vi "SMS Candidate Selection.vi"(0 "Image Ref (U16)":T1, 7 "Blink Sensitivity":sgl=1.3, 11 "Error In":errorcluster) -> (4 "Image Ref (U16) - Dup":T1, 8 "Cadidate Image Ref":T1, 15 "Error Out":errorcluster)   [LabVIEW 2021]
uses:
  <vilib>/vision/Image Controls.llb/IMAQ Image.ctl
  Microscope Modules/SMS Image Preview/SMS Image Preview Type Defs/SMS Image Preview Actions.ctl
  <vilib>/vision/NI_Vision_Development_Module.lvlib
panel:
  out "Image border size out":i32
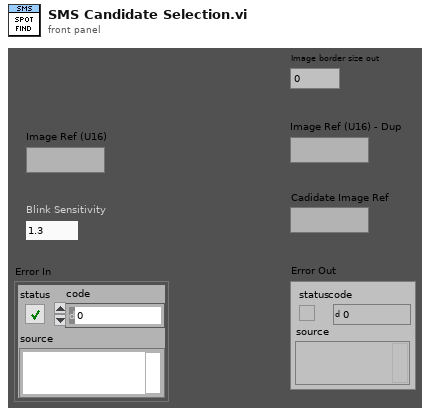
[diagram p1: front panel]
types:
  T1 = typedef "IMAQ Image.ctl" = refnum<image>
  T2 = typedef "Image Type" = u32
  T3 = enum32{"Average", "Min", "Max", "Clear  if < ", "Clear  if < or =", "Clear  if =", "Clear  if > or =", "Clear  if >"}
  T4 = enum32{"AutoM", "Close", "Dilate", "Erode", "Gradient", "Gradient in", "Gradient out", "HitMiss", "Open", "PClose", "POpen", "Thick", "Thin"}
  T5 = cluster{"histogram":u32[], "Minimal Value":sgl, "Maximal Value":sgl, "Starting Value":sgl, "Interval Width":sgl, "Mean Value":sgl, "Standard  Variation":sgl, "Area (pixels)":i32}
  T6 = typedef "SMS Image Preview Actions.ctl" = enum16{"Idle", "Start SMS Preview", "Get Image", "Convolve and Threshold", "Subtract > Dilate", "And Image", "Update Plot", "Abort", "Exit Loop", "Quit"}
  T7 = typedef "SMS Image Preview Notifier Type.ctl" = cluster{"Action":T6, "Camera Notifier Name":string, "Camera Image (U16)":T1, "Camera ROI":cluster{"Global Rectangle":i32[], "Contours":cluster{"Contour Type":u32, "ROI Type":u32, "Points":i32[]}[]}, "SMS Preview (U16)":T1, "Camera ROI (U16)":T1, "Threshold (U16)":T1, "Subtracted > Dilated (U16)":T1, "And Image (U16)":T1, "Camera ROI (SGL)":T1, "Conv 5 x 5 (SGL)":T1, "Conv 11 x 11 (SGL)":T1, "Subtracted (SGL)":T1, "Dilated (SGL)":T1, "Subtracted > Dilated (SGL)":T1, "Ones 5 x 5":sgl[][], "Ones 11 x 11":sgl[][], "Ones 7 x 7":i32[][]}
  T8 = cluster{"Global Rectangle":i32[], "Contours":cluster{"Contour Type":u32, "ROI Type":u32, "Points":i32[]}[]}
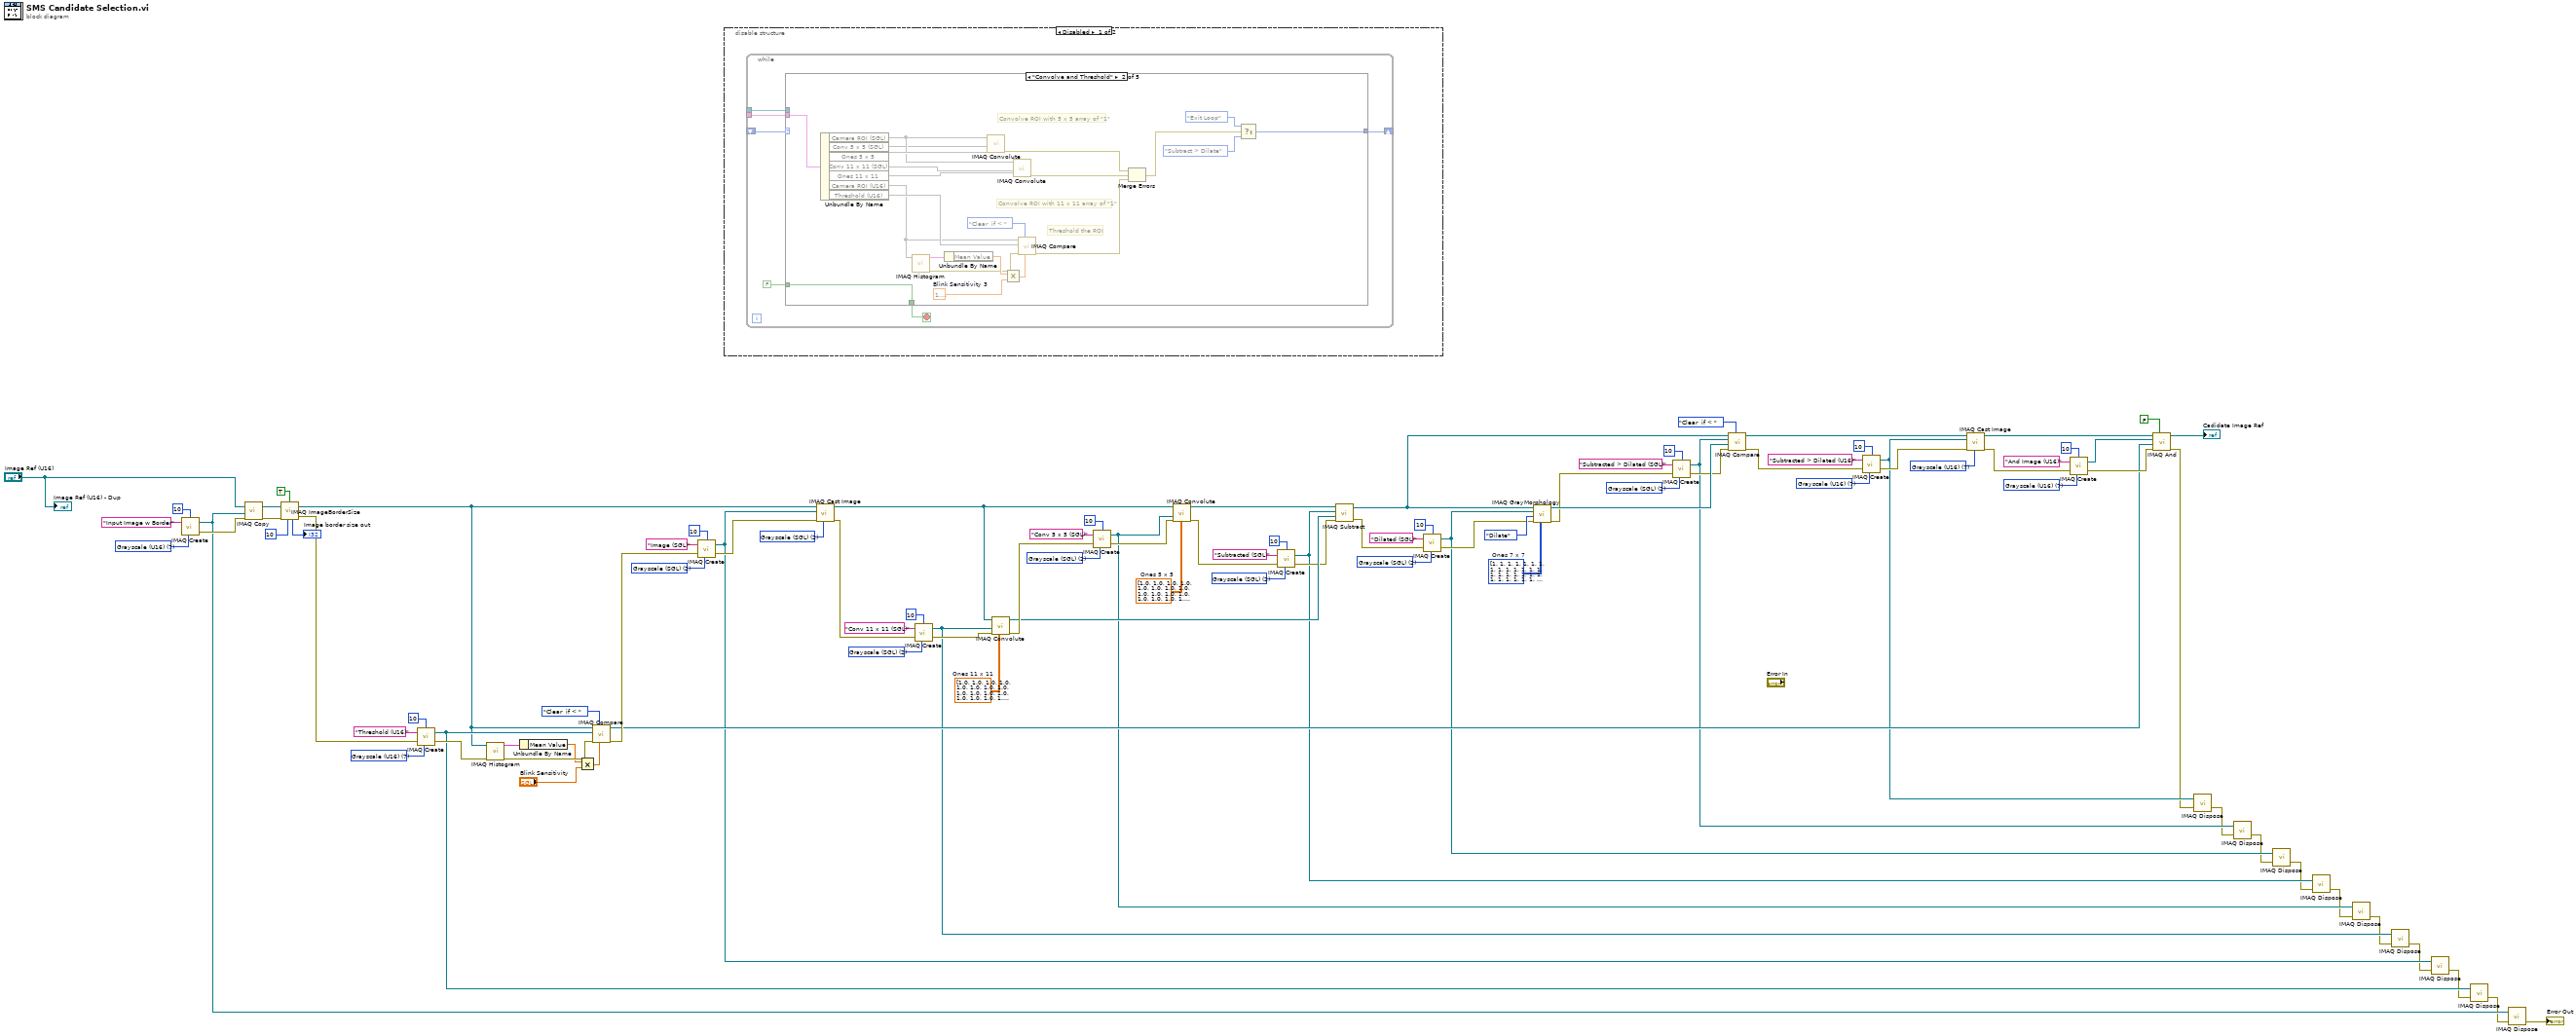
[diagram p0: block diagram]
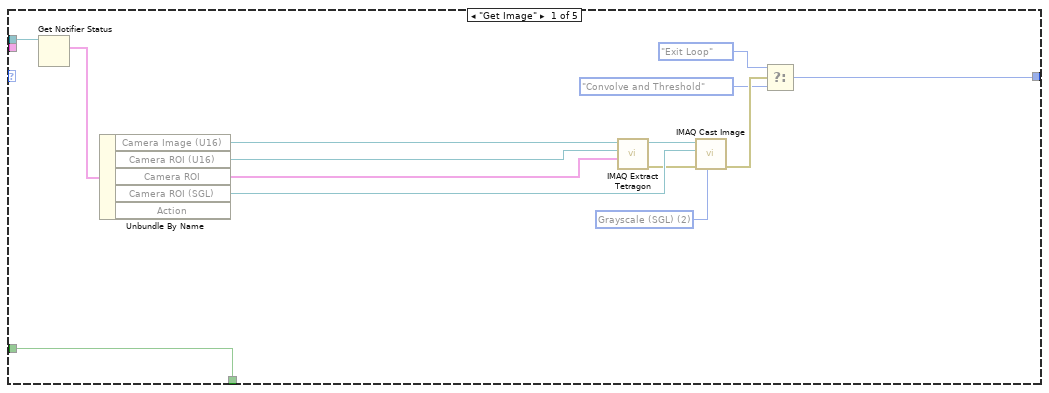
[diagram p2: hidden frame]
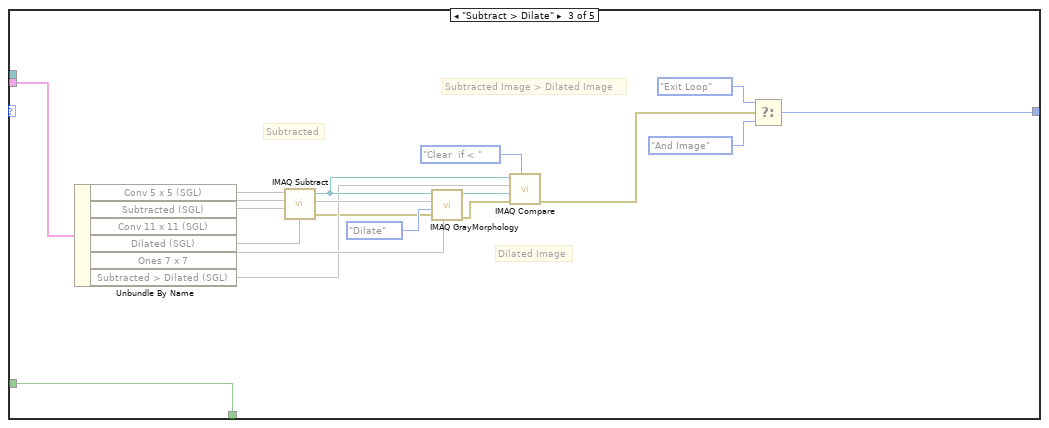
[diagram p3: hidden frame]
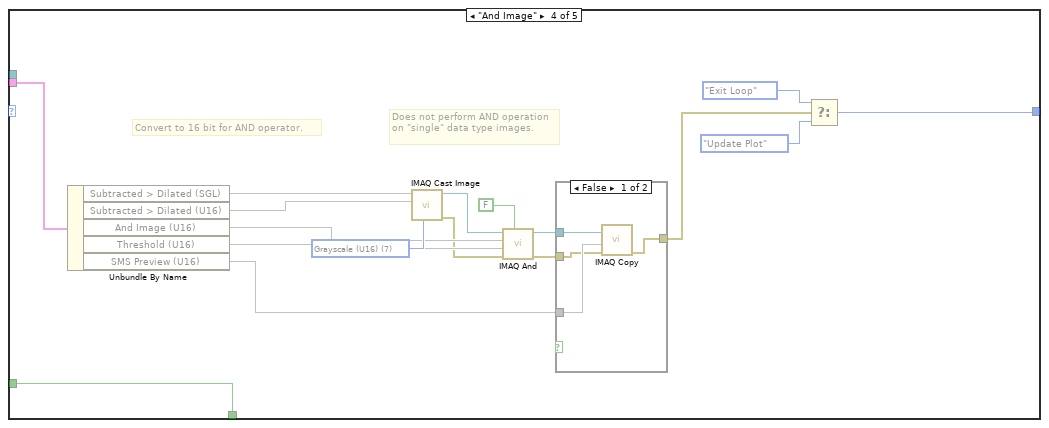
[diagram p4: hidden frame]
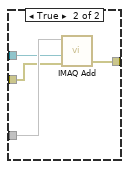
[diagram p5: hidden frame]
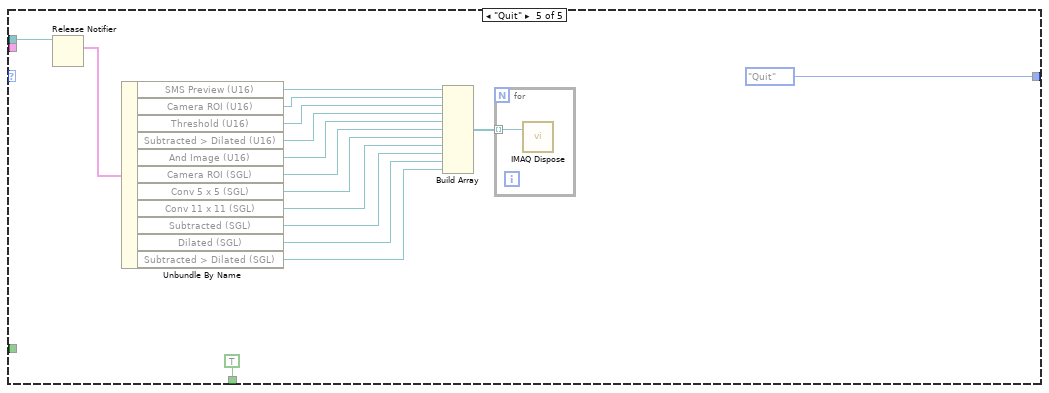
[diagram p6: hidden frame]
diagram:
  w15 = T2 7 items=["Grayscale (U8)", "Grayscale (I16)", "Grayscale (SGL)", "Complex (CSG)", "RGB (U32)", "HSL (U32)", "RGB (U64)", "Grayscale (U16)"] ("Image Type")
  w38 = T2 7 items=["Grayscale (U8)", "Grayscale (I16)", "Grayscale (SGL)", "Complex (CSG)", "RGB (U32)", "HSL (U32)", "RGB (U64)", "Grayscale (U16)"] ("Image Type")
  w48 = T2 7 items=["Grayscale (U8)", "Grayscale (I16)", "Grayscale (SGL)", "Complex (CSG)", "RGB (U32)", "HSL (U32)", "RGB (U64)", "Grayscale (U16)"] ("Image Type")
  w50 = T2 7 items=["Grayscale (U8)", "Grayscale (I16)", "Grayscale (SGL)", "Complex (CSG)", "RGB (U32)", "HSL (U32)", "RGB (U64)", "Grayscale (U16)"] ("Image Type")
  w53 = T2 2 items=["Grayscale (U8)", "Grayscale (I16)", "Grayscale (SGL)", "Complex (CSG)", "RGB (U32)", "HSL (U32)", "RGB (U64)", "Grayscale (U16)"] ("Image Type")
  w59 = i32[][] [[1, 1, 1, 1, 1, 1, 1], [1, 1, 1, 1, 1, 1, 1], [1, 1, 1, 1, 1, 1, 1], [1, 1, 1, 1, 1, 1, 1], [1, 1, 1, 1, 1, 1, 1], [1, 1, 1, 1, 1, 1, 1], [1, 1, 1, 1, 1, 1, 1]]  # Ones 7 x 7
  w63 = T2 2 items=["Grayscale (U8)", "Grayscale (I16)", "Grayscale (SGL)", "Complex (CSG)", "RGB (U32)", "HSL (U32)", "RGB (U64)", "Grayscale (U16)"] ("Image Type")
  w72 = T2 2 items=["Grayscale (U8)", "Grayscale (I16)", "Grayscale (SGL)", "Complex (CSG)", "RGB (U32)", "HSL (U32)", "RGB (U64)", "Grayscale (U16)"] ("Image Type")
  w79 = T2 7 items=["Grayscale (U8)", "Grayscale (I16)", "Grayscale (SGL)", "Complex (CSG)", "RGB (U32)", "HSL (U32)", "RGB (U64)", "Grayscale (U16)"] ("Image Type")
  w89 = T2 2 items=["Grayscale (U8)", "Grayscale (I16)", "Grayscale (SGL)", "Complex (CSG)", "RGB (U32)", "HSL (U32)", "RGB (U64)", "Grayscale (U16)"] ("Image Type")
  w90 = T2 2 items=["Grayscale (U8)", "Grayscale (I16)", "Grayscale (SGL)", "Complex (CSG)", "RGB (U32)", "HSL (U32)", "RGB (U64)", "Grayscale (U16)"] ("Image Type")
  w93 = sgl[][] [[1.0, 1.0, 1.0, 1.0, 1.0, 1.0, 1.0, 1.0, 1.0, 1.0, 1.0], [1.0, 1.0, 1.0, 1.0, 1.0, 1.0, 1.0, 1.0, 1.0, 1.0, 1.0], [1.0, 1.0, 1.0, 1.0, 1.0, 1.0, 1.0, 1.0, 1.0, 1.0, 1.0], [1.0, 1.0, 1.0, 1.0, 1.0, 1.0, 1.0, 1.0, 1.0, 1.0, 1.0], [1.0, 1.0, 1.0, 1.0, 1.0, 1.0, 1.0, 1.0, 1.0, 1.0, 1.0], [1.0, 1.0, 1.0, 1.0, 1.0, 1.0, 1.0, 1.0, 1.0, 1.0, 1.0], [1.0, 1.0, 1.0, 1.0, 1.0, 1.0, 1.0, 1.0, 1.0, 1.0, 1.0], [1.0, 1.0, 1.0, 1.0, 1.0, 1.0, 1.0, 1.0, 1.0, 1.0, 1.0], [1.0, 1.0, 1.0, 1.0, 1.0, 1.0, 1.0, 1.0, 1.0, 1.0, 1.0], [1.0, 1.0, 1.0, 1.0, 1.0, 1.0, 1.0, 1.0, 1.0, 1.0, 1.0], [1.0, 1.0, 1.0, 1.0, 1.0, 1.0, 1.0, 1.0, 1.0, 1.0, 1.0]]  # Ones 11 x 11
  w94 = sgl[][] [[1.0, 1.0, 1.0, 1.0, 1.0], [1.0, 1.0, 1.0, 1.0, 1.0], [1.0, 1.0, 1.0, 1.0, 1.0], [1.0, 1.0, 1.0, 1.0, 1.0], [1.0, 1.0, 1.0, 1.0, 1.0]]  # Ones 5 x 5
  w98 = T2 2 items=["Grayscale (U8)", "Grayscale (I16)", "Grayscale (SGL)", "Complex (CSG)", "RGB (U32)", "HSL (U32)", "RGB (U64)", "Grayscale (U16)"] ("Image Type")
  w99 = T2 2 items=["Grayscale (U8)", "Grayscale (I16)", "Grayscale (SGL)", "Complex (CSG)", "RGB (U32)", "HSL (U32)", "RGB (U64)", "Grayscale (U16)"] ("Image Type")
  n1 = call "IMAQ Create"("Border Size"=10, "Image Name"="Input Image w Border", "Image Type"=w15) -> ("New Image"=w10:T1, "error out"=w12:errorcluster)  [unwired: 2 in]
  n2 = call "IMAQ Copy"("error in (no error)"=w12, "Image Dst"=w10, "Image Src"="Image Ref (U16)") -> ("error out"=w3:errorcluster, "Image Dst Out"=w7:T1)  [unwired: 3 in]
  n3 = call "IMAQ ImageBorderSize"("Get/Set Status? (Set)"=TRUE, "Image"=w7, "Image border size in"=10, "error in (no error)"=w3) -> ("Image Out"=w5:T1, "error out"=w2:errorcluster, "Image border size out"=→"Image border size out":i32)
  n4 = call "IMAQ Create"("Border Size"=10, "Image Name"="Threshold (U16)", "Image Type"=w79, "error in (no error)"=w2) -> ("New Image"=w32:T1, "error out"=w40:errorcluster)  [unwired: 1 in]
  n5 = call "IMAQ Histogram"("error in (no error)"=w40, "Image"=w5) -> ("error out"=w78:errorcluster, "Histogram Report"=w75:T5)  [unwired: 8 in]
  n6 = Unbundle By Name(w75) -> ("Mean Value"=w74:sgl)
  n7 = Multiply(x=w74, y="Blink Sensitivity") -> (x*y=w73:sgl)
  n8 = call "IMAQ Compare"("Constant"=w73, "Operator"=T3."Clear  if < ", "error in (no error)"=w78, "Image Dst"=w32, "Image Src A"=w5) -> ("error out"=w41:errorcluster, "Image Dst Out"=w34:T1)  [unwired: 5 in]
  n9 = call "IMAQ Create"("Border Size"=10, "Image Name"="Image (SGL)", "Image Type"=w98, "error in (no error)"=w41) -> ("New Image"=w31:T1, "error out"=w83:errorcluster)  [unwired: 1 in]
  n10 = disable-structure shown="Disabled" {
    frame Disabled {
      n11 = while {
        shift-right: [w103] -> _
        shift-left: _ -> [w105]
        tunnel: _ -> [w104]
        tunnel: _ -> [w102]
        stop <- w100 stop-if-true
        n12 = case shown="\"Convolve and Threshold\"" w105 {
          tunnel: w104 -> [_ w141 w159 w176 _]
          tunnel: [w110 w122 w142 w160 SMS_Image_Preview_Actions."Quit" ("f")] -> w103
          tunnel: w102 -> [w115 _ _ _ w198]
          tunnel: FALSE -> [w116 w132 w148 w166 _]
          tunnel: [w116 w132 w148 w166 TRUE] -> w100
          frame "Get Image" {
            w108 = T2 2 items=["Grayscale (U8)", "Grayscale (I16)", "Grayscale (SGL)", "Complex (CSG)", "RGB (U32)", "HSL (U32)", "RGB (U64)", "Grayscale (U16)"] ("Image Type")
            n13 = Get Notifier Status(notifier=w115) -> (current notification=w114:T7)  [unwired: 1 in, 4 out]
            n14 = Unbundle By Name(w114) -> ("Camera Image (U16)"=w119:T1, "Camera ROI (U16)"=w118:T1, "Camera ROI"=w117:T8, "Camera ROI (SGL)"=w113:T1)  [unwired: 1 out]
            n15 = call-poly "IMAQ Extract Tetragon"("ROI Descriptor"=w117, "Image Dst"=w118, "Image Src"=w119) -> ("error out"=w106:errorcluster, "Image Dst Out"=w107:T1)  [unwired: 7 in]
            n16 = call "IMAQ Cast Image"("Image Type"=w108, "error in (no error)"=w106, "Image Dst"=w113, "Image Src"=w107) -> ("error out"=w112:errorcluster)  [unwired: 6 in, 1 out]
            n17 = Select(t=SMS_Image_Preview_Actions."Exit Loop", s=w112, f=SMS_Image_Preview_Actions."Convolve and Threshold" ("y")) -> (s? t:f=w110:T6)
          }
          frame "Convolve and Threshold" {
            w128 = sgl 1.3  # Blink Sensitivity 3
            # "Threshold the ROI"
            # "Convolve ROI with 11 x 11 array of \"1\""
            # "Convolve ROI with 5 x 5 array of \"1\""
            n18 = Unbundle By Name(w141) -> ("Camera ROI (SGL)"=w134, "Conv 5 x 5 (SGL)"=w131, "Ones 5 x 5"=w140, "Conv 11 x 11 (SGL)"=w130, "Ones 11 x 11"=w139, "Camera ROI (U16)"=w129, "Threshold (U16)"=w133)
            n19 = call "IMAQ Histogram"("Image"=w129) -> ("error out"=w120:errorcluster, "Histogram Report"=w136:T5)  [unwired: 9 in]
            n20 = Unbundle By Name(w136) -> ("Mean Value"=w137:sgl)
            n21 = call "IMAQ Convolute"("Kernel"=w140, "Image Dst"=w131, "Image Src"=w134) -> ("error out"=w127:errorcluster)  [unwired: 7 in, 1 out]
            n22 = Multiply(x=w137, y=w128) -> (x*y=w138:sgl)
            n23 = call "IMAQ Convolute"("Kernel"=w139, "Image Dst"=w130, "Image Src"=w134) -> ("error out"=w126:errorcluster)  [unwired: 7 in, 1 out]
            n24 = call "IMAQ Compare"("Constant"=w138, "Operator"=T3."Clear  if < ", "error in (no error)"=w120, "Image Dst"=w133, "Image Src A"=w129) -> ("error out"=w125:errorcluster)  [unwired: 5 in, 1 out]
            n25 = Merge Errors(w127, w126, w125) -> (w124:errorcluster)
            n26 = Select(t=SMS_Image_Preview_Actions."Exit Loop", s=w124, f=SMS_Image_Preview_Actions."Subtract > Dilate" ("y")) -> (s? t:f=w122:T6)
          }
          frame "Subtract > Dilate" {
            # "Subtracted Image > Dilated Image"
            # "Subtracted"
            # "Dilated Image"
            n27 = Unbundle By Name(w159) -> ("Conv 5 x 5 (SGL)"=w158, "Subtracted (SGL)"=w157, "Conv 11 x 11 (SGL)"=w156, "Dilated (SGL)"=w153, "Ones 7 x 7"=w154, "Subtracted > Dilated (SGL)"=w149)
            n28 = call "IMAQ Subtract"("Image Src A"=w158, "Image Dst"=w157, "Image Src B"=w156) -> ("Image Dst Out"=w150:T1, "error out"=w147:errorcluster)  [unwired: 4 in]
            n29 = call "IMAQ GrayMorphology"("Structuring Element"=w154, "error in (no error)"=w147, "Operation"=T4."Dilate", "Image Dst"=w153, "Image Src"=w150) -> ("error out"=w146:errorcluster, "Image Dst Out"=w151:T1)  [unwired: 5 in]
            n30 = call "IMAQ Compare"("Operator"=T3."Clear  if < ", "error in (no error)"=w146, "Image Src B"=w151, "Image Dst"=w149, "Image Src A"=w150) -> ("error out"=w145:errorcluster)  [unwired: 5 in, 1 out]
            n31 = Select(t=SMS_Image_Preview_Actions."Exit Loop", s=w145, f=SMS_Image_Preview_Actions."And Image" ("y")) -> (s? t:f=w142:T6)
          }
          frame "And Image" {
            w174 = T2 7 items=["Grayscale (U8)", "Grayscale (I16)", "Grayscale (SGL)", "Complex (CSG)", "RGB (U32)", "HSL (U32)", "RGB (U64)", "Grayscale (U16)"] ("Image Type")
            # "Convert to 16 bit for AND operator."
            # "Does not perform AND operation on \"single\" data type images."
            n32 = Unbundle By Name(w176) -> ("Subtracted > Dilated (SGL)"=w173, "Subtracted > Dilated (U16)"=w172, "And Image (U16)"=w170, "Threshold (U16)"=w169, "SMS Preview (U16)"=w167)
            n33 = call "IMAQ Cast Image"("Image Type"=w174, "Image Dst"=w172, "Image Src"=w173) -> ("error out"=w165:errorcluster, "Image Dst Out"=w171:T1)  [unwired: 7 in]
            n34 = call "IMAQ And"("And/Nand (And)"=FALSE, "error in (no error)"=w165, "Image Src B"=w169, "Image Dst"=w170, "Image Src A"=w171) -> ("error out"=w164:errorcluster, "Image Dst Out"=w168:T1)  [unwired: 5 in]
            n35 = case shown="False" {
              selector: _ -> [_ _]
              tunnel: w168 -> [w180 w183]
              tunnel: w167 -> [w179 w184]
              tunnel: w164 -> [w178 w182]
              tunnel: [w177 w181] -> w161
              frame False {
                n36 = call "IMAQ Copy"("error in (no error)"=w178, "Image Dst"=w179, "Image Src"=w180) -> ("error out"=w177:errorcluster)  [unwired: 3 in, 1 out]
              }
              frame True {
                n37 = call "IMAQ Add"("Image Src A"=w184, "Image Src B"=w183, "error in (no error)"=w182) -> ("error out"=w181:errorcluster)  [unwired: 4 in, 1 out]
              }
            }
            n38 = Select(t=SMS_Image_Preview_Actions."Exit Loop", s=w161, f=SMS_Image_Preview_Actions."Update Plot" ("y")) -> (s? t:f=w160:T6)
          }
          frame "Quit" {
            n39 = Release Notifier(notifier=w198) -> (last notification=w197:T7)  [unwired: 2 in, 2 out]
            n40 = Unbundle By Name(w197) -> ("SMS Preview (U16)"=w196:T1, "Camera ROI (U16)"=w194:T1, "Threshold (U16)"=w193:T1, "Subtracted > Dilated (U16)"=w192:T1, "And Image (U16)"=w191:T1, "Camera ROI (SGL)"=w190:T1, "Conv 5 x 5 (SGL)"=w189:T1, "Conv 11 x 11 (SGL)"=w188:T1, "Subtracted (SGL)"=w187:T1, "Dilated (SGL)"=w186:T1, "Subtracted > Dilated (SGL)"=w185:T1)
            n41 = Build Array(w196, w194, w193, w192, w191, w190, w189, w188, w187, w186, w185) -> (w195:T1[])
            n42 = for {
              tunnel: w195 -> [w201] mode=indexing
              n43 = call "IMAQ Dispose"("Image"=w201) -> ()  [unwired: 5 in, 1 out]
            }
          }
        }
      }
    }
    frame Enabled {
    }
  }
  n44 = call "IMAQ Cast Image"("Image Type"=w99, "error in (no error)"=w83, "Image Dst"=w31, "Image Src"=w5) -> ("error out"=w82:errorcluster, "Image Dst Out"=w95:T1)  [unwired: 6 in]
  n45 = call "IMAQ Create"("Border Size"=10, "Image Name"="Conv 11 x 11 (SGL)", "Image Type"=w89, "error in (no error)"=w82) -> ("New Image"=w30:T1, "error out"=w86:errorcluster)  [unwired: 1 in]
  n46 = call "IMAQ Convolute"("Kernel"=w93, "error in (no error)"=w86, "Image Dst"=w30, "Image Src"=w95) -> ("error out"=w84:errorcluster, "Image Dst Out"=w68:T1)  [unwired: 6 in]
  n47 = call "IMAQ Create"("Border Size"=10, "Image Name"="Conv 5 x 5 (SGL)", "Image Type"=w90, "error in (no error)"=w84) -> ("New Image"=w29:T1, "error out"=w85:errorcluster)  [unwired: 1 in]
  n48 = call "IMAQ Convolute"("Kernel"=w94, "error in (no error)"=w85, "Image Dst"=w29, "Image Src"=w95) -> ("error out"=w67:errorcluster, "Image Dst Out"=w69:T1)  [unwired: 6 in]
  n49 = call "IMAQ Create"("Border Size"=10, "Image Name"="Subtracted (SGL)", "Image Type"=w72, "error in (no error)"=w67) -> ("New Image"=w28:T1, "error out"=w66:errorcluster)  [unwired: 1 in]
  n50 = call "IMAQ Subtract"("Image Src A"=w69, "Image Dst"=w28, "Image Src B"=w68, "error in (no error)"=w66) -> ("Image Dst Out"=w57:T1, "error out"=w61:errorcluster)  [unwired: 3 in]
  n51 = call "IMAQ Create"("Border Size"=10, "Image Name"="Dilated (SGL)", "Image Type"=w63, "error in (no error)"=w61) -> ("New Image"=w27:T1, "error out"=w60:errorcluster)  [unwired: 1 in]
  n52 = call "IMAQ GrayMorphology"("Structuring Element"=w59, "error in (no error)"=w60, "Operation"=T4."Dilate", "Image Dst"=w27, "Image Src"=w57) -> ("error out"=w52:errorcluster, "Image Dst Out"=w56:T1)  [unwired: 5 in]
  n53 = call "IMAQ Create"("Border Size"=10, "Image Name"="Subtracted > Dilated (SGL)", "Image Type"=w53, "error in (no error)"=w52) -> ("New Image"=w26:T1, "error out"=w51:errorcluster)  [unwired: 1 in]
  n54 = call "IMAQ Compare"("Operator"=T3."Clear  if < ", "error in (no error)"=w51, "Image Src B"=w56, "Image Dst"=w26, "Image Src A"=w57) -> ("error out"=w45:errorcluster, "Image Dst Out"=w49:T1)  [unwired: 5 in]
  n55 = call "IMAQ Create"("Border Size"=10, "Image Name"="Subtracted > Dilated (U16)", "Image Type"=w48, "error in (no error)"=w45) -> ("New Image"=w25:T1, "error out"=w44:errorcluster)  [unwired: 1 in]
  n56 = call "IMAQ Cast Image"("Image Type"=w50, "error in (no error)"=w44, "Image Dst"=w25, "Image Src"=w49) -> ("error out"=w36:errorcluster, "Image Dst Out"=w42:T1)  [unwired: 6 in]
  n57 = call "IMAQ Create"("Border Size"=10, "Image Name"="And Image (U16)", "Image Type"=w38, "error in (no error)"=w36) -> ("New Image"=w33:T1, "error out"=w35:errorcluster)  [unwired: 1 in]
  n58 = call "IMAQ And"("And/Nand (And)"=FALSE, "error in (no error)"=w35, "Image Src B"=w34, "Image Dst"=w33, "Image Src A"=w42) -> ("error out"=w16:errorcluster, "Image Dst Out"=→"Cadidate Image Ref":T1)  [unwired: 5 in]
  n59 = call "IMAQ Dispose"("Image"=w25, "error in (no error)"=w16) -> ("error out"=w24:errorcluster)  [unwired: 4 in]
  n60 = call "IMAQ Dispose"("Image"=w26, "error in (no error)"=w24) -> ("error out"=w23:errorcluster)  [unwired: 4 in]
  n61 = call "IMAQ Dispose"("Image"=w27, "error in (no error)"=w23) -> ("error out"=w22:errorcluster)  [unwired: 4 in]
  n62 = call "IMAQ Dispose"("Image"=w28, "error in (no error)"=w22) -> ("error out"=w21:errorcluster)  [unwired: 4 in]
  n63 = call "IMAQ Dispose"("Image"=w29, "error in (no error)"=w21) -> ("error out"=w20:errorcluster)  [unwired: 4 in]
  n64 = call "IMAQ Dispose"("Image"=w30, "error in (no error)"=w20) -> ("error out"=w19:errorcluster)  [unwired: 4 in]
  n65 = call "IMAQ Dispose"("Image"=w31, "error in (no error)"=w19) -> ("error out"=w18:errorcluster)  [unwired: 4 in]
  n66 = call "IMAQ Dispose"("Image"=w32, "error in (no error)"=w18) -> ("error out"=w9:errorcluster)  [unwired: 4 in]
  n67 = call "IMAQ Dispose"("Image"=w10, "error in (no error)"=w9) -> ("error out"=→"Error Out":errorcluster)  [unwired: 4 in]
  "Image Ref (U16) - Dup" <- "Image Ref (U16)"
